vi "SPARK Configure Analog Sensor.vi"   [LabVIEW 2027]
doc: "Configure the analog sensor connected to the data port of the SPARK."
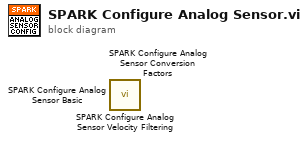
[diagram p0: block diagram]
diagram:
  n1 = call <vilib>:"SPARK Configure Analog Sensor Velocity Filtering.vi"() -> ()  [unwired: 10 in, 2 out]
  n2 = call <vilib>:"SPARK Configure Analog Sensor Conversion Factors.vi"() -> ()  [unwired: 10 in, 2 out]
  n3 = call <vilib>:"SPARK Configure Analog Sensor Basic.vi"() -> ()  [unwired: 10 in, 2 out]
